vi "Delete LVClass from ProjectItem.vi"(7 "Delete Containing Folder?":bool, 8 "error in (no error)":errorcluster, 10 "LV Class Name":string, 11 "ProjectItem in":refnum<vi>) -> (0 "error out":errorcluster, 3 "ProjectItem out":refnum<vi>)   [LabVIEW 2019, in "gRPC Template Creation Utility.lvlib"]
uses:
  gRPC Template Creation Utility.lvlib
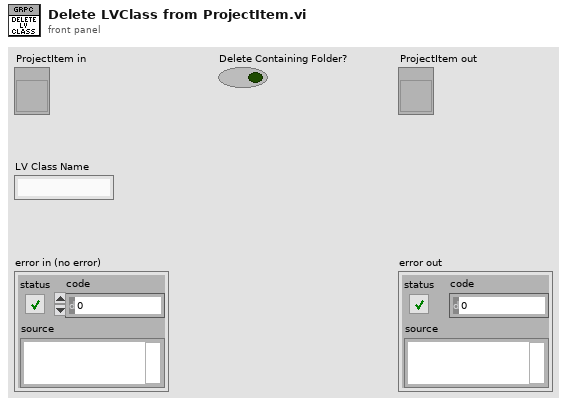
[diagram p1: front panel]
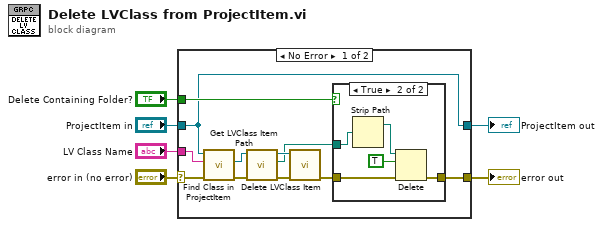
[diagram p0: block diagram]
diagram:
  n1 = case shown="No Error" "error in (no error)" {
    selector: "error in (no error)" -> [w9 w24]
    tunnel: [w17 w24] -> w6
    tunnel: "LV Class Name" -> [w11 _]
    tunnel: "ProjectItem in" -> [w8 w25]
    tunnel: "Delete Containing Folder?" -> [w10 _]
    tunnel: [w8 w25] -> w1
    frame No Error {
      n2 = call "Find Class in ProjectItem.vi"("error in (no error)"=w9, "Class Name"=w11, "ProjectItem in"=w8) -> ("error out"=w13:errorcluster, "LVClass out"=w12:refnum<vi>)  [unwired: 5 in, 2 out]
      n3 = call "Get LVClass Item Path.vi"("error in (no error)"=w13, "LVClassLibrary in"=w12) -> ("error out"=w15:errorcluster, "Path"=w7:path, "LVClassLibrary out"=w14:refnum<vi>)  [unwired: 7 in]
      n4 = call "Delete LVClass Item.vi"("error in (no error)"=w15, "LVClassLibrary in"=w14) -> ("error out"=w16:errorcluster)  [unwired: 9 in]
      n5 = case shown="True" w10 {
        tunnel: [w18 w23] -> w17
        tunnel: w16 -> [w18 w21]
        tunnel: w7 -> [_ w20]
        frame False {
        }
        frame True {
          n6 = Strip Path(path=w20) -> (stripped path=w19:path)  [unwired: 1 out]
          n7 = Delete(path (use dialog)=w19, entire hierarchy (F)=TRUE, error in=w21) -> (error out=w23:errorcluster)  [unwired: 2 in, 2 out]
        }
      }
    }
    frame Error {
    }
  }
  "error out" <- w6
  "ProjectItem out" <- w1
